vi "PicoScopeospaAdvancedTriggerSettings.vi"(0 "handle in":i16=16384, 2 "Trigger holdoff (Samples)":u64, 5 "error in":errorcluster, 6 "Trigger Conditions":T7={"Channel A"=1, "Channel B"=0, "Channel C"=0, "Channel D"=0, "Channel E"=0, "Channel F"=0, "Channel G"=0, "Channel H"=0, "Port 0"=0, "Port 1"=0, "Aux"=0, "PWQ"=0, "Condition Logic"=0} {"Port 1" items=["Don't Care", "True", "False"]; "Channel H" items=["Don't Care", "True", "False"]; "Channel G" items=["Don't Care", "True", "False"]; "Channel F" items=["Don't Care", "True", "False"]; "Channel E" items=["Don't Care", "True", "False"]; "PWQ" items=["Don't Care", "True", "False"]; "Aux" items=["Don't Care", "True", "False"]; "Port 0" items=["Don't Care", "True", "False"]; "Channel D" items=["Don't Care", "True", "False"]; "Channel C" items=["Don't Care", "True", "False"]; "Channel B" items=["Don't Care", "True", "False"]; "Channel A" items=["Don't Care", "True", "False"]; "Condition Logic" items=["AND", "OR", "XOR"]}, 7 "Pulse Width Qualifier Conditions":T1 {"Port 1" items=["Don't Care", "True", "False"]; "Channel H" items=["Don't Care", "True", "False"]; "Channel G" items=["Don't Care", "True", "False"]; "Channel F" items=["Don't Care", "True", "False"]; "Channel E" items=["Don't Care", "True", "False"]; "Aux" items=["Don't Care", "True", "False"]; "Port 0" items=["Don't Care", "True", "False"]; "Channel D" items=["Don't Care", "True", "False"]; "Channel C" items=["Don't Care", "True", "False"]; "Channel B" items=["Don't Care", "True", "False"]; "Channel A" items=["Don't Care", "True", "False"]; "Condition Logic" items=["AND", "OR", "XOR"]}, 8 "Channel Trigger Properties":T5={"Channel A Trigger Properties"={"thresholdUpper"=0, "thresholdUpperHysteresis"=1638, "thresholdLower"=0, "thresholdLowerHysteresis"=1638, "Threshold Mode"=0, "Direction"=2, "Available"=TRUE}, "Channel B Trigger Properties"={"thresholdUpper"=0, "thresholdUpperHysteresis"=1638, "thresholdLower"=0, "thresholdLowerHysteresis"=1638, "Threshold Mode"=0, "Direction"=2, "Available"=FALSE}, "Channel C Trigger Properties"={"thresholdUpper"=0, "thresholdUpperHysteresis"=1638, "thresholdLower"=0, "thresholdLowerHysteresis"=1638, "Threshold Mode"=0, "Direction"=2, "Available"=FALSE}, "Channel D Trigger Properties"={"thresholdUpper"=0, "thresholdUpperHysteresis"=1638, "thresholdLower"=0, "thresholdLowerHysteresis"=1638, "Threshold Mode"=0, "Direction"=2, "Available"=FALSE}, "Channel E Trigger Properties"={"thresholdUpper"=0, "thresholdUpperHysteresis"=0, "thresholdLower"=0, "thresholdLowerHysteresis"=0, "Threshold Mode"=0, "Direction"=2, "Available"=FALSE}, "Channel F Trigger Properties"={"thresholdUpper"=0, "thresholdUpperHysteresis"=0, "thresholdLower"=0, "thresholdLowerHysteresis"=0, "Threshold Mode"=0, "Direction"=2, "Available"=FALSE}, "Channel G Trigger Properties"={"thresholdUpper"=0, "thresholdUpperHysteresis"=0, "thresholdLower"=0, "thresholdLowerHysteresis"=0, "Threshold Mode"=0, "Direction"=2, "Available"=FALSE}, "Channel H Trigger Properties"={"thresholdUpper"=0, "thresholdUpperHysteresis"=0, "thresholdLower"=0, "thresholdLowerHysteresis"=0, "Threshold Mode"=0, "Direction"=2, "Available"=FALSE}} {"Channel H Trigger Properties"."Direction" items=["Above / Inside", "Below / Outside", "Rising / Enter", "Falling / Exit", "Rising or Falling / Enter or Exit", "Above Lower", "Below Lower", "Rising Lower", "Falling Lower", "Positive Runt", "Negative Runt"]; "Channel H Trigger Properties"."Threshold Mode" items=["Level", "Window"]; "Channel G Trigger Properties"."Direction" items=["Above / Inside", "Below / Outside", "Rising / Enter", "Falling / Exit", "Rising or Falling / Enter or Exit", "Above Lower", "Below Lower", "Rising Lower", "Falling Lower", "Positive Runt", "Negative Runt"]; "Channel G Trigger Properties"."Threshold Mode" items=["Level", "Window"]; "Channel F Trigger Properties"."Direction" items=["Above / Inside", "Below / Outside", "Rising / Enter", "Falling / Exit", "Rising or Falling / Enter or Exit", "Above Lower", "Below Lower", "Rising Lower", "Falling Lower", "Positive Runt", "Negative Runt"]; "Channel F Trigger Properties"."Threshold Mode" items=["Level", "Window"]; "Channel E Trigger Properties"."Direction" items=["Above / Inside", "Below / Outside", "Rising / Enter", "Falling / Exit", "Rising or Falling / Enter or Exit", "Above Lower", "Below Lower", "Rising Lower", "Falling Lower", "Positive Runt", "Negative Runt"]; "Channel E Trigger Properties"."Threshold Mode" items=["Level", "Window"]; "Channel D Trigger Properties"."Direction" items=["Above / Inside", "Below / Outside", "Rising / Enter", "Falling / Exit", "Rising or Falling / Enter or Exit", "Above Lower", "Below Lower", "Rising Lower", "Falling Lower", "Positive Runt", "Negative Runt"]; "Channel D Trigger Properties"."Threshold Mode" items=["Level", "Window"]; "Channel C Trigger Properties"."Direction" items=["Above / Inside", "Below / Outside", "Rising / Enter", "Falling / Exit", "Rising or Falling / Enter or Exit", "Above Lower", "Below Lower", "Rising Lower", "Falling Lower", "Positive Runt", "Negative Runt"]; "Channel C Trigger Properties"."Threshold Mode" items=["Level", "Window"]; "Channel B Trigger Properties"."Direction" items=["Above / Inside", "Below / Outside", "Rising / Enter", "Falling / Exit", "Rising or Falling / Enter or Exit", "Above Lower", "Below Lower", "Rising Lower", "Falling Lower", "Positive Runt", "Negative Runt"]; "Channel B Trigger Properties"."Threshold Mode" items=["Level", "Window"]; "Channel A Trigger Properties"."Direction" items=["Above / Inside", "Below / Outside", "Rising / Enter", "Falling / Exit", "Rising or Falling / Enter or Exit", "Above Lower", "Below Lower", "Rising Lower", "Falling Lower", "Positive Runt", "Negative Runt"]; "Channel A Trigger Properties"."Threshold Mode" items=["Level", "Window"]}, 9 "Pulse Width Qualifier Trigger Properties":T2={"Channel A Trigger Properties"={"Threshold Mode"=0, "Available"=TRUE, "Direction"=2}, "Channel B Trigger Properties"={"Threshold Mode"=0, "Available"=FALSE, "Direction"=2}, "Channel C Trigger Properties"={"Threshold Mode"=0, "Available"=FALSE, "Direction"=2}, "Channel D Trigger Properties"={"Threshold Mode"=0, "Available"=FALSE, "Direction"=2}, "Channel E Trigger Properties"={"Threshold Mode"=0, "Available"=FALSE, "Direction"=2}, "Channel F Trigger Properties"={"Threshold Mode"=0, "Available"=FALSE, "Direction"=2}, "Channel G Trigger Properties"={"Threshold Mode"=0, "Available"=FALSE, "Direction"=2}, "Channel H Trigger Properties"={"Threshold Mode"=0, "Available"=FALSE, "Direction"=2}, "Port 0 Trigger Properties"={"Threshold Mode"=0, "Available"=FALSE, "Direction"=2}, "Port 1 Trigger Properties"={"Threshold Mode"=0, "Available"=FALSE, "Direction"=2}} {"Port 1 Trigger Properties"."Direction" items=["Rising"=2, "Falling"=3, "Rising Lower"=7, "Above"=0, "Below"=1, "Rising or Falling"=4, "Falling Lower"=8, "Below Lower"=6, "Above Lower"=5]; "Port 1 Trigger Properties"."Threshold Mode" items=["Level", "Window"]; "Port 0 Trigger Properties"."Direction" items=["Rising"=2, "Falling"=3, "Rising Lower"=7, "Above"=0, "Below"=1, "Rising or Falling"=4, "Falling Lower"=8, "Below Lower"=6, "Above Lower"=5]; "Port 0 Trigger Properties"."Threshold Mode" items=["Level", "Window"]; "Channel H Trigger Properties"."Direction" items=["Rising"=2, "Falling"=3, "Rising Lower"=7, "Above"=0, "Below"=1, "Rising or Falling"=4, "Falling Lower"=8, "Below Lower"=6, "Above Lower"=5]; "Channel H Trigger Properties"."Threshold Mode" items=["Level", "Window"]; "Channel G Trigger Properties"."Direction" items=["Rising"=2, "Falling"=3, "Rising Lower"=7, "Above"=0, "Below"=1, "Rising or Falling"=4, "Falling Lower"=8, "Below Lower"=6, "Above Lower"=5]; "Channel G Trigger Properties"."Threshold Mode" items=["Level", "Window"]; "Channel F Trigger Properties"."Direction" items=["Rising"=2, "Falling"=3, "Rising Lower"=7, "Above"=0, "Below"=1, "Rising or Falling"=4, "Falling Lower"=8, "Below Lower"=6, "Above Lower"=5]; "Channel F Trigger Properties"."Threshold Mode" items=["Level", "Window"]; "Channel E Trigger Properties"."Direction" items=["Rising"=2, "Falling"=3, "Rising Lower"=7, "Above"=0, "Below"=1, "Rising or Falling"=4, "Falling Lower"=8, "Below Lower"=6, "Above Lower"=5]; "Channel E Trigger Properties"."Threshold Mode" items=["Level", "Window"]; "Channel D Trigger Properties"."Direction" items=["Rising"=2, "Falling"=3, "Rising Lower"=7, "Above"=0, "Below"=1, "Rising or Falling"=4, "Falling Lower"=8, "Below Lower"=6, "Above Lower"=5]; "Channel D Trigger Properties"."Threshold Mode" items=["Level", "Window"]; "Channel C Trigger Properties"."Direction" items=["Rising"=2, "Falling"=3, "Rising Lower"=7, "Above"=0, "Below"=1, "Rising or Falling"=4, "Falling Lower"=8, "Below Lower"=6, "Above Lower"=5]; "Channel C Trigger Properties"."Threshold Mode" items=["Level", "Window"]; "Channel B Trigger Properties"."Direction" items=["Rising"=2, "Falling"=3, "Rising Lower"=7, "Above"=0, "Below"=1, "Rising or Falling"=4, "Falling Lower"=8, "Below Lower"=6, "Above Lower"=5]; "Channel B Trigger Properties"."Threshold Mode" items=["Level", "Window"]; "Channel A Trigger Properties"."Direction" items=["Rising"=2, "Falling"=3, "Rising Lower"=7, "Above"=0, "Below"=1, "Rising or Falling"=4, "Falling Lower"=8, "Below Lower"=6, "Above Lower"=5]; "Channel A Trigger Properties"."Threshold Mode" items=["Level", "Window"]}, 10 "Digital Ports":T4 {"Digital Port  1"."Direction Channel 15" items=["Don't Care", "Low", "High", "Rising", "Falling"]; "Digital Port  1"."Direction Channel 14" items=["Don't Care", "Low", "High", "Rising", "Falling"]; "Digital Port  1"."Direction Channel 13" items=["Don't Care", "Low", "High", "Rising", "Falling"]; "Digital Port  1"."Direction Channel 12" items=["Don't Care", "Low", "High", "Rising", "Falling"]; "Digital Port  1"."Direction Channel 11" items=["Don't Care", "Low", "High", "Rising", "Falling"]; "Digital Port  1"."Direction Channel 10" items=["Don't Care", "Low", "High", "Rising", "Falling"]; "Digital Port  1"."Direction Channel 9" items=["Don't Care", "Low", "High", "Rising", "Falling"]; "Digital Port  1"."Direction Channel 8" items=["Don't Care", "Low", "High", "Rising", "Falling"]; "Digital Port  0"."Direction Channel 7" items=["Don't Care", "Low", "High", "Rising", "Falling"]; "Digital Port  0"."Direction Channel 6" items=["Don't Care", "Low", "High", "Rising", "Falling"]; "Digital Port  0"."Direction Channel 5" items=["Don't Care", "Low", "High", "Rising", "Falling"]; "Digital Port  0"."Direction Channel 4" items=["Don't Care", "Low", "High", "Rising", "Falling"]; "Digital Port  0"."Direction Channel 3" items=["Don't Care", "Low", "High", "Rising", "Falling"]; "Digital Port  0"."Direction Channel 2" items=["Don't Care", "Low", "High", "Rising", "Falling"]; "Digital Port  0"."Direction Channel 1" items=["Don't Care", "Low", "High", "Rising", "Falling"]; "Digital Port  0"."Direction Channel 0" items=["Don't Care", "Low", "High", "Rising", "Falling"]}, 11 "Pulse Width Qualifier Settings":T3 {"Pulse Width Type" items=["None", "Less Than", "Greater Than", "In Range", "Out of Range"]}, 12 "Auto Trigger (us)":u32=1000000 format="%.4p", 13 "Trigger Delay (samples)":u64) -> (14 "handle out":i16=16384, 19 "error out":errorcluster)   [LabVIEW 2010]
doc: "This VI is an interface for the advanced trigger features of the oscilloscope.\nA simple trigger can be set using PicoScopeXXXXSettings.vi, in which case it is not necessary to use this VI."
uses:
  psospa.dll
panel:
  in  "Addition Trigger Properties":T6={"Ext. Trigger Properties (DO NOT USE)"={"thresholdUpper"=0, "thresholdUpperHysteresis"=0, "thresholdLower"=0, "thresholdLowerHysteresis"=0, "Threshold Mode"=0, "Direction"=2, "Available"=FALSE}, "Aux. Trigger Properties"={"thresholdUpper"=0, "thresholdUpperHysteresis"=0, "thresholdLower"=0, "thresholdLowerHysteresis"=0, "Threshold Mode"=0, "Direction"=2, "Available"=FALSE}} {"Aux. Trigger Properties"."Direction" items=["Above / Inside", "Below / Outside", "Rising / Enter", "Falling / Exit", "Rising or Falling / Enter or Exit", "Above Lower", "Below Lower", "Rising Lower", "Falling Lower", "Positive Runt", "Negative Runt"]; "Aux. Trigger Properties"."Threshold Mode" items=["Level", "Window"]; "Ext. Trigger Properties (DO NOT USE)"."Direction" items=["Above / Inside", "Below / Outside", "Rising / Enter", "Falling / Exit", "Rising or Falling / Enter or Exit", "Above Lower", "Below Lower", "Rising Lower", "Falling Lower", "Positive Runt", "Negative Runt"]; "Ext. Trigger Properties (DO NOT USE)"."Threshold Mode" items=["Level", "Window"]}
  in  "SetTrigger Info Action XOR":bool=TRUE
  out "XOR Debug Array":u32[][](array[numeric])
  in  "SetTrigger Info Action OR":bool=TRUE
  # "For Condition Logic Suggested settings;\nFor AND, XOR logic-(parallel triggers)\nUse level-type triggers (Level or Inside/outside Window Triggers)\n\nFor OR logic- (single channel)\nUse edge types (e.g. rising, falling, entering window)"
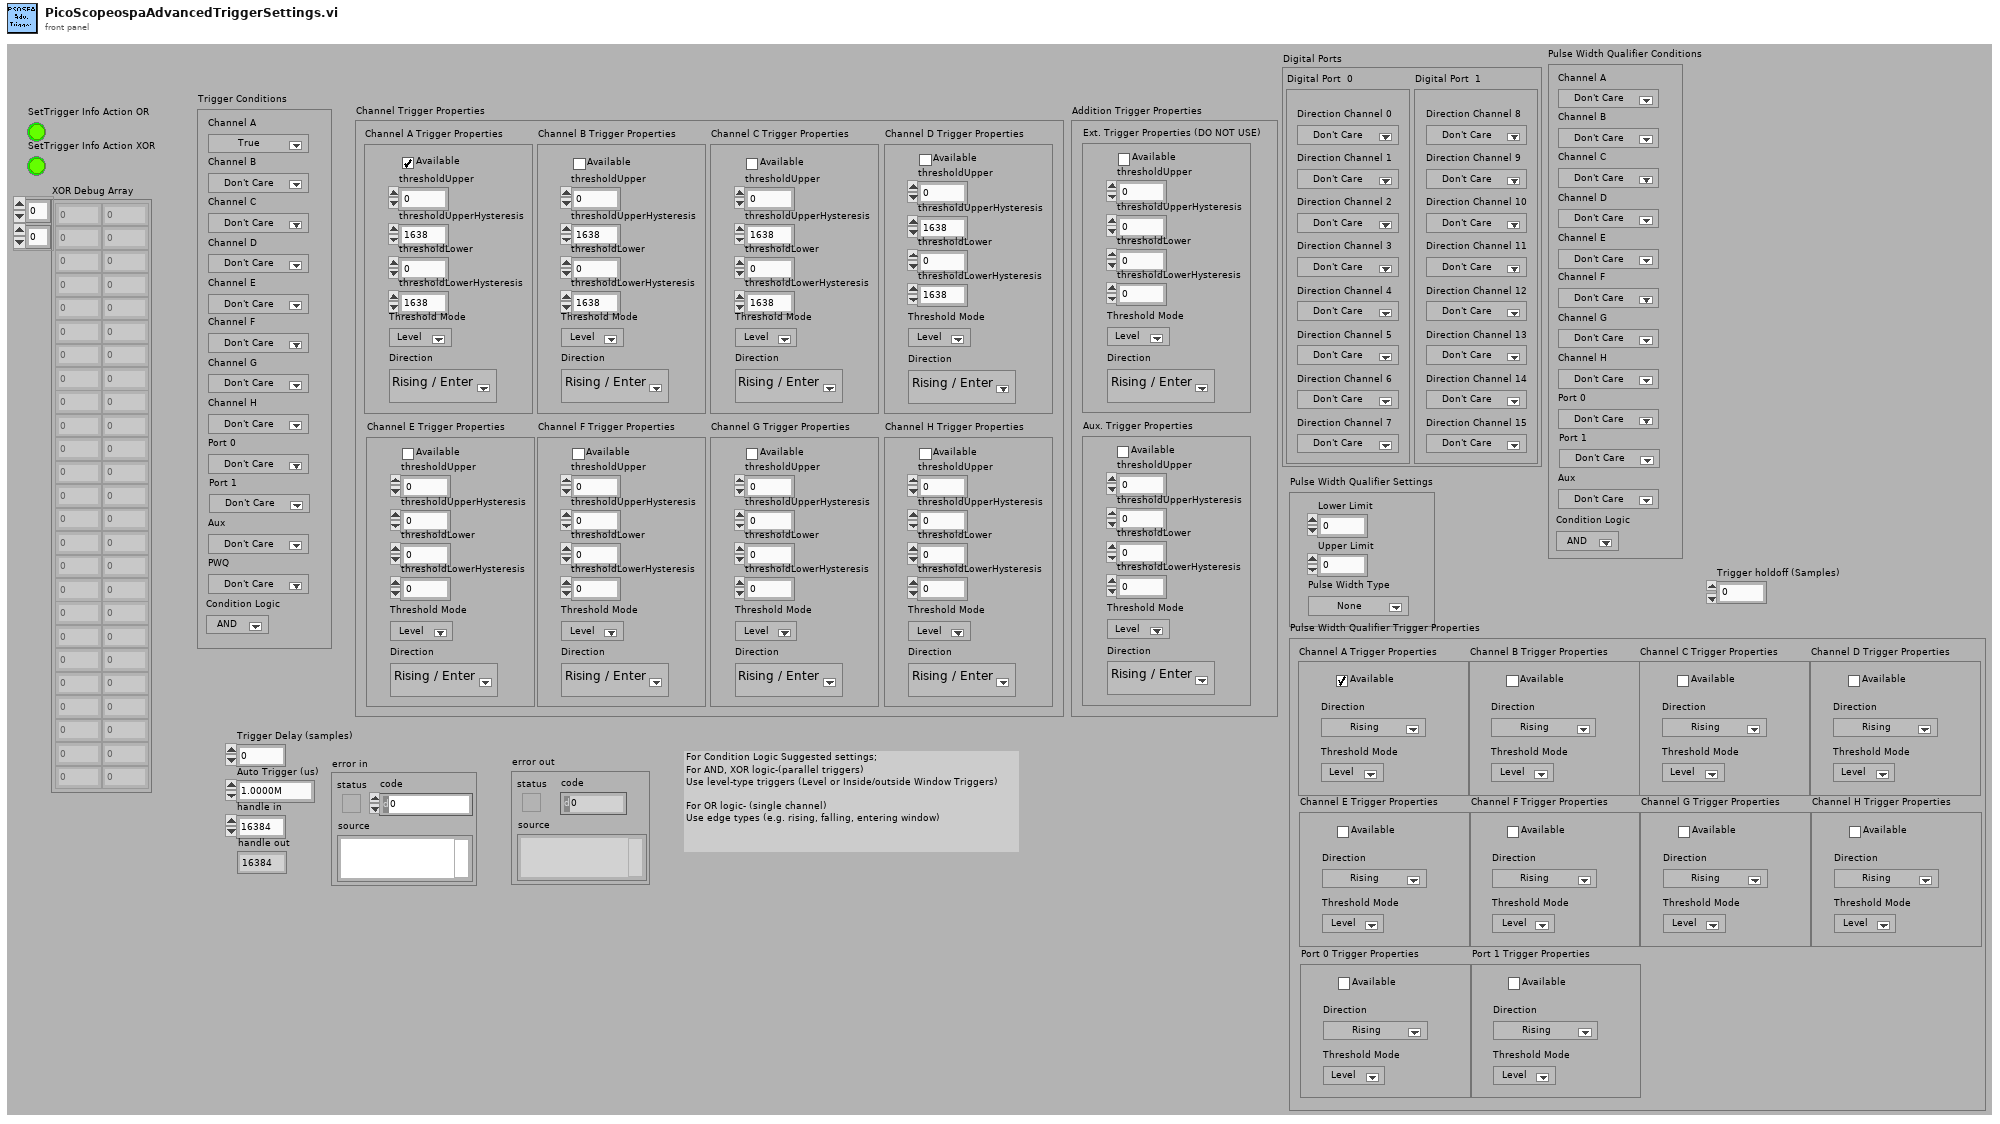
[diagram p1: front panel]
types:
  T1 = cluster{"Channel A":u16, "Channel B":u16, "Channel C":u16, "Channel D":u16, "Channel E":u16, "Channel F":u16, "Channel G":u16, "Channel H":u16, "Port 0":u16, "Port 1":u16, "Aux":u16, "Condition Logic":u16}
  T2 = cluster{"Channel A Trigger Properties":cluster{"Threshold Mode":i32, "Available":bool, "Direction":u32}, "Channel B Trigger Properties":cluster{"Threshold Mode":i32, "Available":bool, "Direction":u32}, "Channel C Trigger Properties":cluster{"Threshold Mode":i32, "Available":bool, "Direction":u32}, "Channel D Trigger Properties":cluster{"Threshold Mode":i32, "Available":bool, "Direction":u32}, "Channel E Trigger Properties":cluster{"Threshold Mode":i32, "Available":bool, "Direction":u32}, "Channel F Trigger Properties":cluster{"Threshold Mode":i32, "Available":bool, "Direction":u32}, "Channel G Trigger Properties":cluster{"Threshold Mode":i32, "Available":bool, "Direction":u32}, "Channel H Trigger Properties":cluster{"Threshold Mode":i32, "Available":bool, "Direction":u32}, "Port 0 Trigger Properties":cluster{"Threshold Mode":i32, "Available":bool, "Direction":u32}, "Port 1 Trigger Properties":cluster{"Threshold Mode":i32, "Available":bool, "Direction":u32}}
  T3 = cluster{"Lower Limit":u32, "Upper Limit":u32, "Pulse Width Type":u32}
  T4 = cluster{"Digital Port  0":cluster{"Direction Channel 0":u16, "Direction Channel 1":u16, "Direction Channel 2":u16, "Direction Channel 3":u16, "Direction Channel 4":u16, "Direction Channel 5":u16, "Direction Channel 6":u16, "Direction Channel 7":u16}, "Digital Port  1":cluster{"Direction Channel 8":u16, "Direction Channel 9":u16, "Direction Channel 10":u16, "Direction Channel 11":u16, "Direction Channel 12":u16, "Direction Channel 13":u16, "Direction Channel 14":u16, "Direction Channel 15":u16}}
  T5 = cluster{"Channel A Trigger Properties":cluster{"thresholdUpper":i16, "thresholdUpperHysteresis":u16, "thresholdLower":i16, "thresholdLowerHysteresis":u16, "Threshold Mode":i32, "Direction":i32, "Available":bool}, "Channel B Trigger Properties":cluster{"thresholdUpper":i16, "thresholdUpperHysteresis":u16, "thresholdLower":i16, "thresholdLowerHysteresis":u16, "Threshold Mode":i32, "Direction":i32, "Available":bool}, "Channel C Trigger Properties":cluster{"thresholdUpper":i16, "thresholdUpperHysteresis":u16, "thresholdLower":i16, "thresholdLowerHysteresis":u16, "Threshold Mode":i32, "Direction":i32, "Available":bool}, "Channel D Trigger Properties":cluster{"thresholdUpper":i16, "thresholdUpperHysteresis":u16, "thresholdLower":i16, "thresholdLowerHysteresis":u16, "Threshold Mode":i32, "Direction":i32, "Available":bool}, "Channel E Trigger Properties":cluster{"thresholdUpper":i16, "thresholdUpperHysteresis":u16, "thresholdLower":i16, "thresholdLowerHysteresis":u16, "Threshold Mode":i32, "Direction":i32, "Available":bool}, "Channel F Trigger Properties":cluster{"thresholdUpper":i16, "thresholdUpperHysteresis":u16, "thresholdLower":i16, "thresholdLowerHysteresis":u16, "Threshold Mode":i32, "Direction":i32, "Available":bool}, "Channel G Trigger Properties":cluster{"thresholdUpper":i16, "thresholdUpperHysteresis":u16, "thresholdLower":i16, "thresholdLowerHysteresis":u16, "Threshold Mode":i32, "Direction":i32, "Available":bool}, "Channel H Trigger Properties":cluster{"thresholdUpper":i16, "thresholdUpperHysteresis":u16, "thresholdLower":i16, "thresholdLowerHysteresis":u16, "Threshold Mode":i32, "Direction":i32, "Available":bool}}
  T6 = cluster{"Ext. Trigger Properties (DO NOT USE)":cluster{"thresholdUpper":i16, "thresholdUpperHysteresis":u16, "thresholdLower":i16, "thresholdLowerHysteresis":u16, "Threshold Mode":i32, "Direction":i32, "Available":bool}, "Aux. Trigger Properties":cluster{"thresholdUpper":i16, "thresholdUpperHysteresis":u16, "thresholdLower":i16, "thresholdLowerHysteresis":u16, "Threshold Mode":i32, "Direction":i32, "Available":bool}}
  T7 = cluster{"Channel A":u16, "Channel B":u16, "Channel C":u16, "Channel D":u16, "Channel E":u16, "Channel F":u16, "Channel G":u16, "Channel H":u16, "Port 0":u16, "Port 1":u16, "Aux":u16, "PWQ":u16, "Condition Logic":u16}
  T8 = cluster{"thresholdUpper":i16, "thresholdUpperHysteresis":u16, "thresholdLower":i16, "thresholdLowerHysteresis":u16, "Threshold Mode":i32, "Direction":i32, "Available":bool}[]
  T9 = cluster{"status":bool, "code":u32, "source":string}
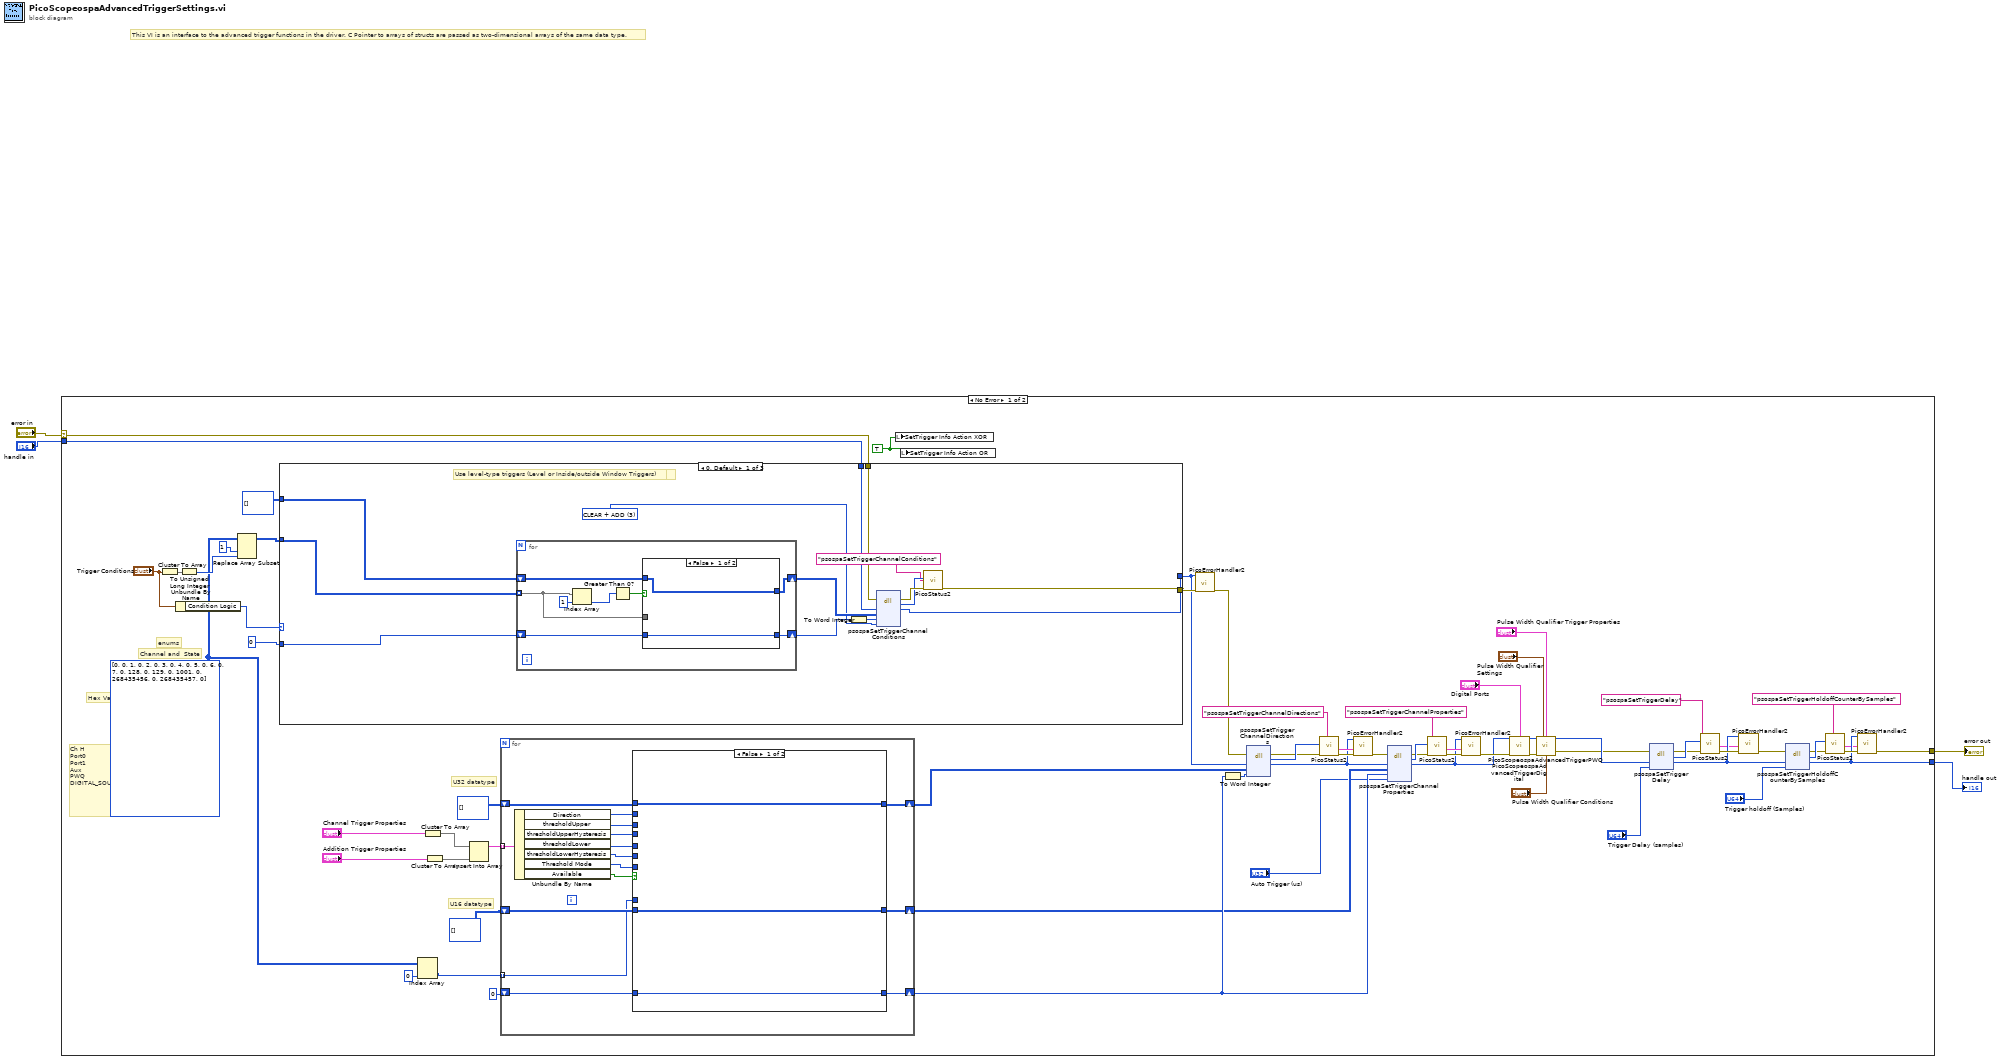
[diagram p0: block diagram]
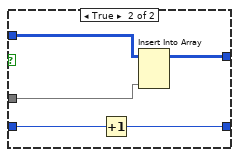
[diagram p2: hidden frame]
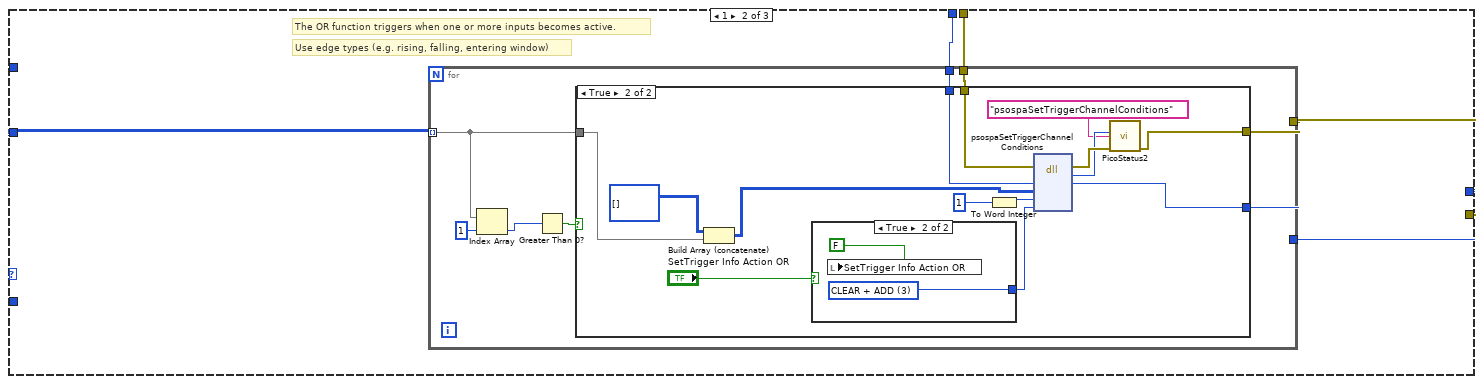
[diagram p3: hidden frame]
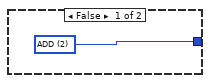
[diagram p5: hidden frame]
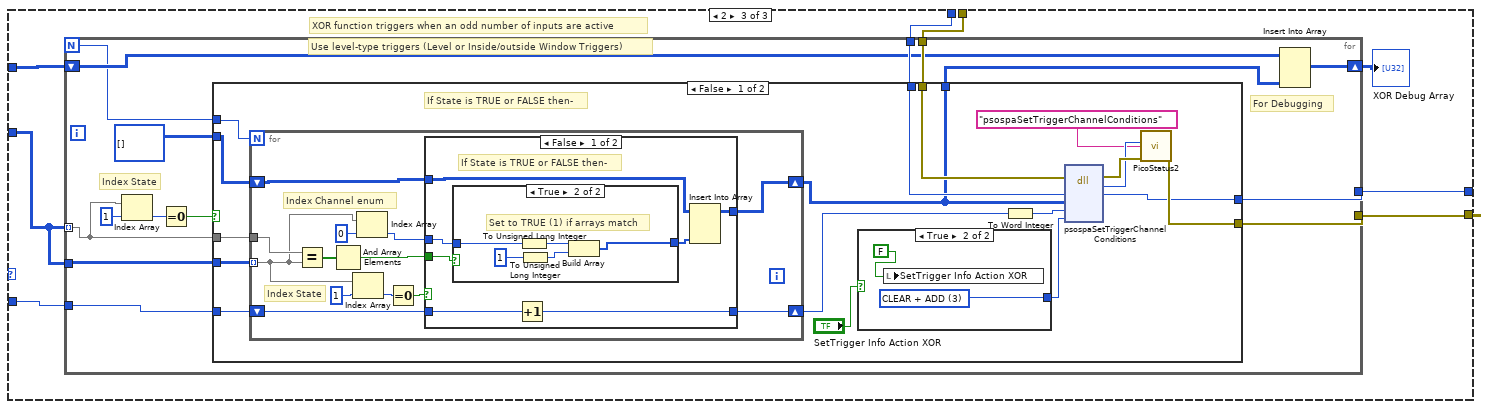
[diagram p6: hidden frame]
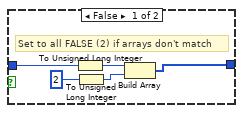
[diagram p7: hidden frame]
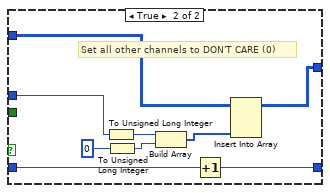
[diagram p8: hidden frame]
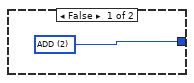
[diagram p9: hidden frame]
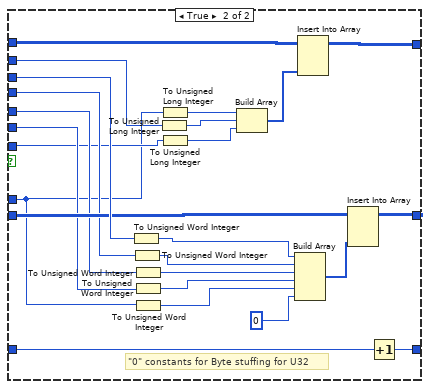
[diagram p11: hidden frame]
diagram:
  # "This VI is an interface to the advanced trigger functions in the driver. C Pointer to arrays of structs are passed as two-dimensional arrays of the same data type."
  n1 = case shown="No Error" "error in" {
    selector: "error in" -> [w44 w261]
    tunnel: "handle in" -> [w43 w262]
    tunnel: [w18 w262] -> w2
    tunnel: [w17 w261] -> w1
    frame No Error {
      w49 = TRUE ("Boolean")
      w34 = u32[][] [[0, 0], [1, 0], [2, 0], [3, 0], [4, 0], [5, 0], [6, 0], [7, 0], [128, 0], [129, 0], [1001, 0], [268435456, 0], [268435457, 0]]
      # "enums"
      # "Ch H\nPort0\nPort1\nAux\nPWQ\nDIGITAL_SOURCE"
      # "Channel and  State"
      # "Hex Values"
      # "U16 datatype"
      # "U32 datatype"
      n2 = Cluster To Array(cluster="Trigger Conditions") -> (array=w55:u16[])
      n3 = Unbundle By Name("Trigger Conditions") -> ("Condition Logic"=w36:u16)
      n4 = To Unsigned Long Integer(number=w55) -> (unsigned 32bit integer=w52:u32[])
      n5 = Replace Array Subset(array=w34, new element=w52, index (col)=1 ("disabled index (col)")) -> (w48:u32[][])  [unwired: 1 in]
      n6 = case shown="0, Default" w36 {
        tunnel: u32[][] [] -> [w86 _ w137]
        tunnel: i16 0 -> [w85 _ w134]
        tunnel: w44 -> [w79 w106 w141]
        tunnel: w43 -> [w78 w105 w140]
        tunnel: [w75 w104 w139] -> w46
        tunnel: [w74 w103 w138] -> w45
        tunnel: w48 -> [w73 w102 w135]
        frame 0, Default {
          w76 = u32 3 items=["CLEAR + ADD"=3, "CLEAR"=1, "ADD"=2] ("Condition Action")
          # "AND function requires both inputs to be active before it will trigger."
          # "Use level-type triggers (Level or Inside/outside Window Triggers)"
          n7 = for {
            shift-right: [w93] -> w81
            shift-left: w85 -> [w92]
            shift-right: [w91] -> w77
            shift-left: w86 -> [w94]
            tunnel: w73 -> [w89] mode=indexing
            n8 = Index Array(array=w89, index=1) -> (element=w88:u32)
            n9 = Greater Than 0?(x=w88) -> (x > 0?=w90:bool)
            n10 = case shown="False" w90 {
              tunnel: w94 -> [w96 w101]
              tunnel: [w96 w100] -> w91
              tunnel: [w95 w99] -> w93
              tunnel: w92 -> [w95 w98]
              tunnel: w89 -> [_ w97]
              frame False {
              }
              frame True {
                n11 = Increment(x=w98) -> (x+1=w99:i16)
                n12 = Insert Into Array(array=w101, new element=w97) -> (w100:u32[][])  [unwired: 2 in]
              }
            }
          }
          n13 = To Word Integer(number=w81) -> (16bit integer=w84:i16)
          n14 = dll-call lib="psospa.dll" fn="psospaSetTriggerChannelConditions" ("ps3000.dll:_ps3000_open_unit@0")(error in=w79, "handle"=w78, "conditions"=w77, "nConditions"=w84, "info"=w76) -> (error out=w83:errorcluster, "PICO_STATUS"=w82:u32, "handle"=w74:i16)  [unwired: 5 in, 1 out]
          n15 = call "PicoStatus2.vi"("PICO source"="psospaSetTriggerChannelConditions" ("source"), "Error in"=w83, "PICO STATUS"=w82) -> ("error out"=w75:errorcluster)  [unwired: 5 in, 1 out]
        }
        frame 1 {
          # "Use edge types (e.g. rising, falling, entering window)"
          # "The OR function triggers when one or more inputs becomes active."
          n16 = for {
            tunnel: w106 -> [w114]
            tunnel: w105 -> [w113]
            tunnel: [w112] -> w104
            tunnel: [w111] -> w103
            tunnel: w102 -> [w109] mode=indexing
            n17 = Index Array(array=w109, index=1) -> (element=w108:u32)
            n18 = Greater Than 0?(x=w108) -> (x > 0?=w107:bool)
            n19 = case shown="True" w107 {
              tunnel: w114 -> [w115 w126]
              tunnel: w113 -> [w116 w125]
              tunnel: [w115 w123] -> w112
              tunnel: [w116 w122] -> w111
              tunnel: w109 -> [_ w117]
              frame False {
              }
              frame True {
                n20 = Build Array (concatenate)(u32[][] [], w117) -> (w119:u32[][])
                n21 = case shown="True" "SetTrigger Info Action OR" {
                  tunnel: [w131 w133] -> w124
                  frame False {
                    w131 = u32 2 items=["CLEAR"=1, "ADD"=2, "CLEAR + ADD"=3] ("Condition Action")
                  }
                  frame True {
                    w133 = u32 3 items=["CLEAR"=1, "ADD"=2, "CLEAR + ADD"=3] ("Condition Action")
                    n22 = local write "SetTrigger Info Action OR"(FALSE ("Boolean")) -> ()
                  }
                }
                n23 = To Word Integer(number=i16 1) -> (16bit integer=w130:i16)
                n24 = dll-call lib="psospa.dll" fn="psospaSetTriggerChannelConditions" ("ps3000.dll:_ps3000_open_unit@0")(error in=w126, "handle"=w125, "conditions"=w119, "nConditions"=w130, "info"=w124) -> (error out=w129:errorcluster, "PICO_STATUS"=w128:u32, "handle"=w122:i16)  [unwired: 5 in, 1 out]
                n25 = call "PicoStatus2.vi"("PICO source"="psospaSetTriggerChannelConditions" ("source"), "Error in"=w129, "PICO STATUS"=w128) -> ("error out"=w123:errorcluster)  [unwired: 5 in, 1 out]
              }
            }
          }
        }
        frame 2 {
          # "Use level-type triggers (Level or Inside/outside Window Triggers)"
          # "XOR function triggers when an odd number of inputs are active"
          n26 = for {
            N -> [w149]
            tunnel: w141 -> [w156]
            tunnel: w140 -> [w155]
            tunnel: [w154] -> w139
            tunnel: [w153] -> w138
            shift-right: [w151] -> w136
            shift-left: w137 -> [w152]
            tunnel: w135 -> [w143] mode=indexing
            tunnel: w135 -> [w146]
            tunnel: w134 -> [w147]
            # "Index State"
            # "For Debugging"
            n27 = Index Array(array=w143, index=1) -> (element=w144:u32)
            n28 = Equal To 0?(x=w144) -> (x = 0?=w142:bool)
            n29 = case shown="False" w142 {
              tunnel: w156 -> [w173 w216]
              tunnel: w155 -> [w172 w217]
              tunnel: [w171 w216] -> w154
              tunnel: [w170 w217] -> w153
              tunnel: [w168 w218] -> w150
              tunnel: w149 -> [w167 _]
              tunnel: u32[][] [] -> [w166 w218]
              tunnel: w147 -> [w165 _]
              tunnel: w146 -> [w164 _]
              tunnel: w143 -> [w163 _]
              frame False {
                # "If State is TRUE or FALSE then-"
                n30 = for {
                  N: w167 -> [_]
                  shift-right: [w185] -> w169
                  shift-left: w165 -> [w186]
                  shift-right: [w174] -> w168
                  shift-left: w166 -> [w175]
                  tunnel: w163 -> [w182]
                  tunnel: w164 -> [w178] mode=indexing
                  # "Index State"
                  # "Index Channel enum"
                  n31 = Equal?(x=w182, y=w178) -> (x = y?=w176:bool[])
                  n32 = And Array Elements(Boolean array=w176) -> (logical AND=w181:bool)
                  n33 = Index Array(array=w178, index=1) -> (element=w179:u32)
                  n34 = Index Array(array=w178, index=0) -> (element=w183:u32)
                  n35 = Equal To 0?(x=w179) -> (x = 0?=w177:bool)
                  n36 = case shown="False" w177 {
                    tunnel: w186 -> [w193 w204]
                    tunnel: [w192 w205] -> w185
                    tunnel: w183 -> [w191 w208]
                    tunnel: w181 -> [w190 _]
                    tunnel: w175 -> [w189 w207]
                    tunnel: [w187 w206] -> w174
                    frame False {
                      # "If State is TRUE or FALSE then-"
                      n37 = case shown="True" w190 {
                        tunnel: [w198 w203] -> w188
                        tunnel: w191 -> [w197 w202]
                        frame False {
                          # "Set to all FALSE (2) if arrays don't match"
                          n38 = To Unsigned Long Integer(number=w197) -> (unsigned 32bit integer=w195:u32)
                          n39 = To Unsigned Long Integer(number=u32 2) -> (unsigned 32bit integer=w196:u32)
                          n40 = Build Array(w195, w196) -> (w198:u32[])
                        }
                        frame True {
                          # "Set to TRUE (1) if arrays match"
                          n41 = To Unsigned Long Integer(number=w202) -> (unsigned 32bit integer=w200:u32)
                          n42 = To Unsigned Long Integer(number=u32 1) -> (unsigned 32bit integer=w201:u32)
                          n43 = Build Array(w200, w201) -> (w203:u32[])
                        }
                      }
                      n44 = Increment(x=w193) -> (x+1=w192:i16)
                      n45 = Insert Into Array(array=w189, new element=w188) -> (w187:u32[][])  [unwired: 2 in]
                    }
                    frame True {
                      # "Set all other channels to DON'T CARE (0)"
                      n46 = To Unsigned Long Integer(number=w208) -> (unsigned 32bit integer=w210:u32)
                      n47 = To Unsigned Long Integer(number=u32 0) -> (unsigned 32bit integer=w211:u32)
                      n48 = Build Array(w210, w211) -> (w212:u32[])
                      n49 = Increment(x=w204) -> (x+1=w205:i16)
                      n50 = Insert Into Array(array=w207, new element=w212) -> (w206:u32[][])  [unwired: 2 in]
                    }
                  }
                }
                n51 = case shown="True" "SetTrigger Info Action XOR" {
                  tunnel: [w213 w215] -> w157
                  frame False {
                    w213 = u32 2 items=["CLEAR + ADD"=3, "CLEAR"=1, "ADD"=2] ("Condition Action")
                  }
                  frame True {
                    w215 = u32 3 items=["CLEAR + ADD"=3, "CLEAR"=1, "ADD"=2] ("Condition Action")
                    n52 = local write "SetTrigger Info Action XOR"(FALSE ("Boolean")) -> ()
                  }
                }
                n53 = To Word Integer(number=w169) -> (16bit integer=w162:i16)
                n54 = dll-call lib="psospa.dll" fn="psospaSetTriggerChannelConditions" ("ps3000.dll:_ps3000_open_unit@0")(error in=w173, "handle"=w172, "conditions"=w168, "nConditions"=w162, "info"=w157) -> (error out=w161:errorcluster, "PICO_STATUS"=w160:u32, "handle"=w170:i16)  [unwired: 5 in, 1 out]
                n55 = call "PicoStatus2.vi"("PICO source"="psospaSetTriggerChannelConditions" ("source"), "Error in"=w161, "PICO STATUS"=w160) -> ("error out"=w171:errorcluster)  [unwired: 5 in, 1 out]
              }
              frame True {
              }
            }
            n56 = Insert Into Array(array=w152, new element=w150) -> (w151:u32[][])  [unwired: 2 in]
          }
          "XOR Debug Array" <- w136
        }
      }
      n57 = Index Array(array=w34, index (col)=0 ("disabled index (col)")) -> (element=w33:u32[])  [unwired: 1 in]
      n58 = Cluster To Array(cluster="Channel Trigger Properties") -> (array=w40:T8)
      n59 = Cluster To Array(cluster="Addition Trigger Properties") -> (array=w38:T8)
      n60 = Insert Into Array(array=w40, new element=w38) -> (w39:T8)  [unwired: 1 in]
      n61 = for {
        tunnel: w39 -> [w220] mode=indexing
        shift-right: [w227] -> w57
        shift-left: i16 0 -> [w226]
        shift-right: [w224] -> w53
        shift-left: u16[][] [] -> [w225]
        shift-right: [w223] -> w54
        shift-left: u32[][] [] -> [w222]
        tunnel: w33 -> [w219] mode=indexing
        n62 = Unbundle By Name(w220) -> ("Direction"=w221:i32, "thresholdUpper"=w233:i16, "thresholdUpperHysteresis"=w232:u16, "thresholdLower"=w231:i16, "thresholdLowerHysteresis"=w230:u16, "Threshold Mode"=w229:i32, "Available"=w228:bool)
        n63 = case shown="False" w228 {
          tunnel: w233 -> [_ w260]
          tunnel: w232 -> [_ w246]
          tunnel: w231 -> [_ w245]
          tunnel: w230 -> [_ w244]
          tunnel: w229 -> [_ w241]
          tunnel: w219 -> [_ w238]
          tunnel: [w236 w259] -> w227
          tunnel: w226 -> [w236 w258]
          tunnel: [w235 w256] -> w224
          tunnel: w225 -> [w235 w255]
          tunnel: [w234 w254] -> w223
          tunnel: w222 -> [w234 w253]
          tunnel: w221 -> [_ w237]
          frame False {
          }
          frame True {
            # "\"0\" constants for Byte stuffing for U32"
            n64 = To Unsigned Word Integer(number=w260) -> (unsigned 16bit integer=w248:u16)
            n65 = To Unsigned Word Integer(number=w246) -> (unsigned 16bit integer=w247:u16)
            n66 = To Unsigned Word Integer(number=w245) -> (unsigned 16bit integer=w243:u16)
            n67 = To Unsigned Word Integer(number=w244) -> (unsigned 16bit integer=w249:u16)
            n68 = To Unsigned Word Integer(number=w238) -> (unsigned 16bit integer=w240:u16)
            n69 = To Unsigned Long Integer(number=w237) -> (unsigned 32bit integer=w251:u32)
            n70 = To Unsigned Long Integer(number=w238) -> (unsigned 32bit integer=w250:u32)
            n71 = To Unsigned Long Integer(number=w241) -> (unsigned 32bit integer=w242:u32)
            n72 = Build Array(w250, w251, w242) -> (w252:u32[])
            n73 = Build Array(w248, w247, w243, w249, w240, u16 0 ("element")) -> (w257:u16[])
            n74 = Insert Into Array(array=w253, new element=w252) -> (w254:u32[][])  [unwired: 2 in]
            n75 = Insert Into Array(array=w255, new element=w257) -> (w256:u16[][])  [unwired: 2 in]
            n76 = Increment(x=w258) -> (x+1=w259:i16)
          }
        }
      }
      n77 = local write "SetTrigger Info Action XOR"(w49) -> ()
      n78 = local write "SetTrigger Info Action OR"(w49) -> ()
      n79 = call "PicoErrorHandler2.vi"("error in (no error)"=w46, "handle In"=w45) -> ("error out"=w51:errorcluster)  [unwired: 9 in]
      n80 = To Word Integer(number=w57) -> (16bit integer=w58:i16)
      n81 = dll-call lib="psospa.dll" fn="psospaSetTriggerChannelDirections" ("ps3000.dll:_ps3000_open_unit@0")(error in=w51, "handle"=w45, "directions"=w54, "nDirections"=w58) -> (error out=w71:errorcluster, "PICO_STATUS"=w72:u32, "handle"=w5:i16)  [unwired: 4 in, 1 out]
      n82 = call "PicoStatus2.vi"("PICO source"="psospaSetTriggerChannelDirections" ("source"), "Error in"=w71, "PICO STATUS"=w72) -> ("error out"=w9:errorcluster, "PICO_STATUS out"=w7:T9)  [unwired: 5 in]
      n83 = call "PicoErrorHandler2.vi"("error in (no error)"=w9, "PICO_STATUS in"=w7, "handle In"=w5) -> ("error out"=w8:errorcluster)  [unwired: 8 in]
      n84 = dll-call lib="psospa.dll" fn="psospaSetTriggerChannelProperties" ("ps3000.dll:_ps3000_open_unit@0")(error in=w8, "handle"=w5, "channelProperties"=w53, "nChannelProperties"=w57, "autoTriggerMicroSeconds"="Auto Trigger (us)") -> (error out=w69:errorcluster, "PICO_STATUS"=w70:u32, "handle"=w6:i16)  [unwired: 5 in, 1 out]
      n85 = call "PicoStatus2.vi"("PICO source"="psospaSetTriggerChannelProperties" ("source"), "Error in"=w69, "PICO STATUS"=w70) -> ("error out"=w12:errorcluster, "PICO_STATUS out"=w10:T9)  [unwired: 5 in]
      n86 = call "PicoErrorHandler2.vi"("error in (no error)"=w12, "PICO_STATUS in"=w10, "handle In"=w6) -> ("error out"=w11:errorcluster)  [unwired: 8 in]
      n87 = call "PicoScopeospaAdvancedTriggerDigital.vi"("handle in"=w6, "Digital Ports"="Digital Ports", "error in"=w11) -> ("handle out"=w32:i16, "error out"=w31:errorcluster)  [unwired: 11 in]
      n88 = call "PicoScopeospaAdvancedTriggerPWQ.vi"("handle in"=w32, "Pulse Width Qualifier Settings"="Pulse Width Qualifier Settings", "Pulse Width Qualifier Trigger Properties"="Pulse Width Qualifier Trigger Properties", "error in"=w31, "Pulse Width Qualifier Conditions"="Pulse Width Qualifier Conditions") -> ("handle out"=w30:i16, "error out"=w29:errorcluster)  [unwired: 9 in]
      n89 = dll-call lib="psospa.dll" fn="psospaSetTriggerDelay" ("ps3000.dll:_ps3000_open_unit@0")(error in=w29, "handle"=w30, "delay"="Trigger Delay (samples)") -> (error out=w67:errorcluster, "PICO_STATUS"=w68:u32, "handle"=w19:i16)  [unwired: 3 in, 1 out]
      n90 = call "PicoStatus2.vi"("PICO source"="psospaSetTriggerDelay" ("source"), "Error in"=w67, "PICO STATUS"=w68) -> ("error out"=w66:errorcluster, "PICO_STATUS out"=w13:T9)  [unwired: 5 in]
      n91 = call "PicoErrorHandler2.vi"("error in (no error)"=w66, "PICO_STATUS in"=w13, "handle In"=w19) -> ("error out"=w20:errorcluster)  [unwired: 8 in]
      n92 = dll-call lib="psospa.dll" fn="psospaSetTriggerHoldoffCounterBySamples" ("ps3000.dll:_ps3000_open_unit@0")(error in=w20, "handle"=w19, "holdoffSamples"="Trigger holdoff (Samples)") -> (error out=w23:errorcluster, "PICO_STATUS"=w24:u32, "handle"=w18:i16)  [unwired: 3 in, 1 out]
      n93 = call "PicoStatus2.vi"("PICO source"="psospaSetTriggerHoldoffCounterBySamples" ("source"), "Error in"=w23, "PICO STATUS"=w24) -> ("error out"=w22:errorcluster, "PICO_STATUS out"=w14:T9)  [unwired: 5 in]
      n94 = call "PicoErrorHandler2.vi"("error in (no error)"=w22, "PICO_STATUS in"=w14, "handle In"=w18) -> ("error out"=w17:errorcluster)  [unwired: 8 in]
    }
    frame Error {
    }
  }
  "handle out" <- w2
  "error out" <- w1
